vi "ZM-HWM-evaluateError.vi"(8 "error in (no error)":errorcluster, 10 "stop actor? in":bool=TRUE, 11 "ZM-HWM-hardware_manager in":refnum<class "ZM-HWM-hardware_manager.lvclass">) -> (0 "error out":errorcluster, 2 "stop actor? out":bool=TRUE, 3 "ZM-HWM-hardware_manager out":refnum<class "ZM-HWM-hardware_manager.lvclass">)   [LabVIEW 2020, in "ZM-HWM-hardware_manager.lvlib" / "ZM-HWM-hardware_manager.lvclass"]
doc: "Error hook of the hardware manager, called by Handle Error and after the helper loop. For now a pass-through: the class, the error and stop actor? go out unchanged; nothing is logged or cleared. Error-handling plan: none yet; an error stops the actor and, through its Last Ack, its caller."
uses:
  ZM-HWM-hardware_manager.lvclass
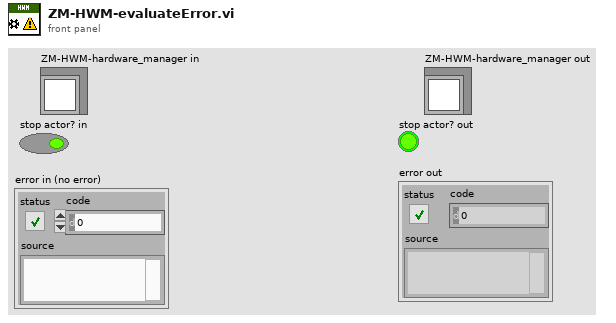
[diagram p1: front panel]
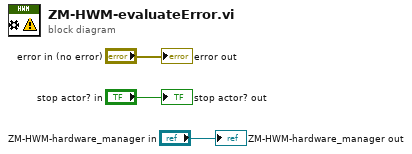
[diagram p0: block diagram]
diagram:
  "ZM-HWM-hardware_manager out" <- "ZM-HWM-hardware_manager in"
  "stop actor? out" <- "stop actor? in"
  "error out" <- "error in (no error)"
